vi "Debug ReadWrite JSON in UTF16-LE.vi"() -> ()   [LabVIEW 2019]
doc: "- - -\nCopyright (c) 2026, Merecs Engineering GmbH"
uses:
  Language Selection/TypeDefs/Cluster Language Configuration.ctl
  Language Selection/community/Cluster Settings Data.ctl
  Language Selection/TypeDefs/Cluster Language.ctl
  Language Selection/TypeDefs/Cluster PropertyTranslation.ctl
  Language Selection/TypeDefs/Enum Property Type.ctl
  Language Selection/private/Hex-String To String.vi
  <vilib>/addons/Tools/Unicode/_subVIs/Convert ASCII to UTF-16LE (Scalar).vi
  <vilib>/addons/Tools/Unicode/Convert UTF-16LE to ASCII.vi
  <vilib>/addons/Tools/Unicode/_subVIs/Convert UTF-16LE to ASCII (Scalar).vi
  <vilib>/addons/Tools/Unicode/UI Unicode Tools.lvlib
  Language Selection/Language Selection.lvlib
  <vilib>/addons/Tools/Unicode/UTF8 Tools.lvlib
  <vilib>/JDP Science/JSONtext/JSONtext.lvlib
panel:
  out "writing text in file":string
  out "Compare Write Read Cluster":bool
  in  "Config Data":T1
  out "String out 2":string="2143B4304394344200310\",\"2143B4304394344200320"
  out "String out":string
  out "<JSON>":string
  in  "Translation":string="!\u0004;\u00040\u00049\u00044\u0004; !\u0004;\u00040\u00049\u00044\u0004 \u00002\u0000"
  out "var to data":string
  out "Unicode":string
  out "UTF-8 Text":string
  # "Ergebnisvergleich nach der Konvertierung von UTF16-LE.\nAchtung: Bei Translation muss \"Force Unicode Text\" aktiviert sein."
  # "UTF16-LE Text wird for der Konvertierung mit JSON text in \"HEX String\" umgewandelt. Hier wird die Konvertierung getestet."
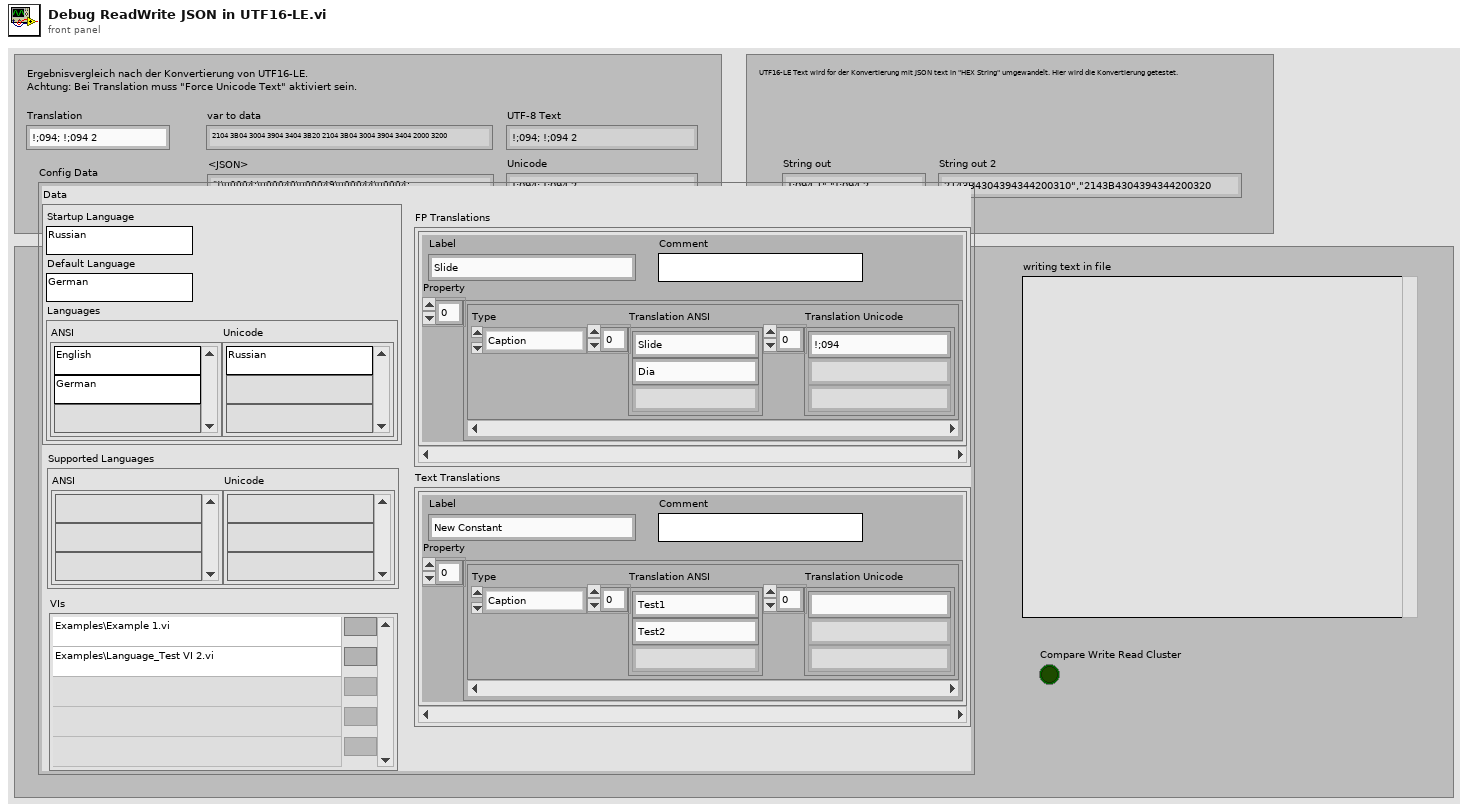
[diagram p1: front panel]
types:
  T1 = typedef "Language Selection.lvlib/Cluster Language Configuration.ctl" = cluster{"Data":T2, "Supported Languages":cluster{"ANSI":string[], "Unicode":string[]}, "VIs":path[], "FP Translations":T3[], "Text Translations":T3[]}
  T2 = typedef "Language Selection.lvlib/Cluster Settings Data.ctl" = cluster{"Startup Language":string, "Default Language":string, "Languages":cluster{"ANSI":string[], "Unicode":string[]}}
  T3 = typedef "Language Selection.lvlib/Cluster Language.ctl" = cluster{"Label":string, "Comment":string, "Property":T4[]}
  T4 = typedef "Language Selection.lvlib/Cluster PropertyTranslation.ctl" = cluster{"Type":T5, "Translation ANSI":string[], "Translation Unicode":string[]}
  T5 = typedef "Language Selection.lvlib/Enum Property Type.ctl" = enum16{"NA", "Caption", "String Value", "Boolean Text", "Ring Strings", "1D Array Elements", "2D Array Elements", "(MC)Listbox Header", "(MC)Listbox Items", "Tab Pages Names", "X & Y GraphChart", "Plot Names", "Table Headers", "Table Items", "TipStrip", "Combobox Strings", "Cursor Name", "Tree Col Headers"}
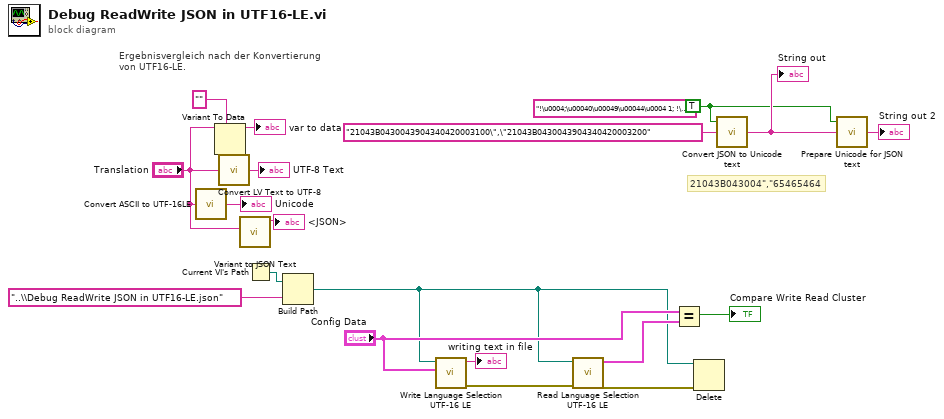
[diagram p0: block diagram]
diagram:
  w7 = TRUE ("Unicode (True)")
  (unwired) "!\u0004;\u00040\u00049\u00044\u0004 1; !\u0004;\u00040\u00049\u00044\u0004 2 " ("Translation")
  # "21043B043004\",\"65465464"
  # "Ergebnisvergleich nach der Konvertierung von UTF16-LE."
  n1 = call-poly <vilib>:"Convert ASCII to UTF-16LE.vi"("ASCII"="Translation") -> ("Unicode"=→"Unicode":string)  [unwired: 4 in]
  n2 = Variant To Data(type="", Variant="Translation") -> (data=→"var to data":string)  [unwired: 1 in, 1 out]
  n3 = call <vilib>:"Convert LV Text to UTF-8.vi"("LV Text"="Translation") -> ("UTF-8 Text"=→"UTF-8 Text":string)  [unwired: 13 in, 1 out]
  n4 = call <vilib>:"Variant to JSON Text.vi"("Variant"="Translation") -> ("<JSON>"=→"<JSON>":string)  [unwired: 8 in, 2 out]
  n5 = Current VI's Path() -> (path=w4:path)
  n6 = Build Path(base path=w4, name or relative path="..\\Debug ReadWrite JSON in UTF16-LE.json") -> (appended path=w2:path)
  n7 = call "Write Language Selection UTF-16 LE.vi"("Langúage Selection"="Config Data", "LanguageSelection file"=w2) -> ("error out"=w9:errorcluster, "text"=→"writing text in file":string)  [unwired: 8 in]
  n8 = call "Read Language Selection UTF-16 LE.vi"("error in (no error)"=w9, "LanguageSelection file"=w2) -> ("error out"=w1:errorcluster, "Language Selection"=w5:T1)  [unwired: 8 in]
  n9 = Equal?(x="Config Data", y=w5) -> (x = y?=→"Compare Write Read Cluster":bool)
  n10 = Delete(path (use dialog)=w2, error in=w1) -> ()  [unwired: 3 in, 3 out]
  n11 = call "Convert JSON to Unicode text.vi"("String in"="21043B0430043904340420003100\",\"21043B0430043904340420003200", "Unicode (True)"=w7) -> ("String out"=w13:string)  [unwired: 3 in]
  "String out" <- w13
  n12 = call "Prepare Unicode for JSON text.vi"("String in"=w13, "Unicode (True)"=w7) -> ("String out"=→"String out 2":string)  [unwired: 3 in]
